vi "Reset.vi"(8 "error in":errorcluster, 11 "Actor in":refnum<class "CounterActor.lvclass">) -> (0 "error out":errorcluster, 3 "Actor out":refnum<class "CounterActor.lvclass">)   [LabVIEW 2026, in "CounterActor.lvclass"]
doc: "Message Counter actor method: Reset. Counter and Processed are private actor state."
uses:
  CounterActor.lvclass
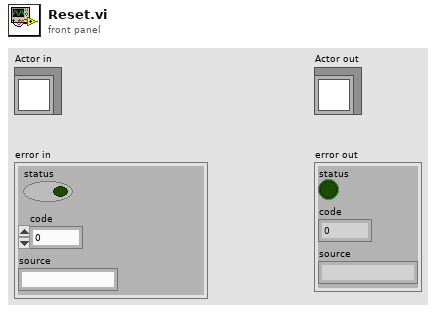
[diagram p1: front panel]
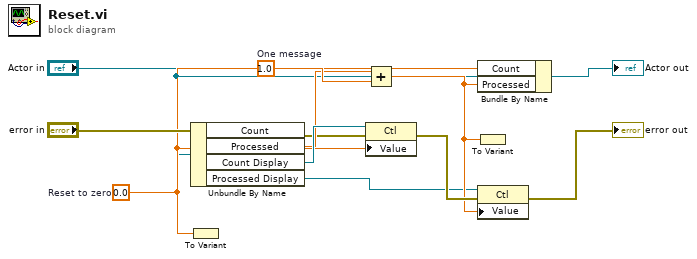
[diagram p0: block diagram]
diagram:
  w7 = 1.0  # One message
  w2 = 0.0  # Reset to zero
  n1 = Unbundle By Name("Actor in") -> ("Processed"=w4:dbl, "Count Display"=w5:refnum<vi>, "Processed Display"=w6:refnum<vi>)  [unwired: 1 out]
  n2 = To Variant(anything=w2) -> ()  [unwired: 1 out]
  n3 = Add(x=w4, y=w7) -> (x+y=w8:dbl)
  n4 = property class="Ctl"(reference=w5, error in="error in", "Value"=w2) -> (error out=w10:errorcluster)  [unwired: 1 out]
  n5 = Bundle By Name(cluster="Actor in", "Count"=w2, "Processed"=w8) -> (→"Actor out":refnum<class "CounterActor.lvclass">)
  n6 = To Variant(anything=w8) -> ()  [unwired: 1 out]
  n7 = property class="Ctl"(reference=w6, error in=w10, "Value"=w8) -> (error out=→"error out":errorcluster)  [unwired: 1 out]
